vi "BSM Signal Table Save.vi"(5 "Base Ex Info":T4, 6 "Total assembly C":T1 {"Assembly Ratio 2" format="%#_3g"; "Assembly Ratio" format="%#_3g"}, 7 "BNAL Path":T2, 8 "error in":errorcluster caption="エラー入力", 9 "Save CV":T5, 10 "BC1":cluster{"B region#":i32, "Date":string}, 11 "LS Path":T3) -> (0 "error out":errorcluster)   [LabVIEW 2018]
panel:
  out "Long Signal#":i32
  out "B region#":i32
  out "L Time Profile Table":string[][](table) caption="Time Table"
  out "LS_E_J Path":path
  out "LS_E_T Path":path
  out "Time Graph":cluster{"time":dbl[], "current":dbl[]}[](graph)
  out "File F_Name":string
  out "LS_T":string
  out "Mx Right Read Seq":i32
  out "T IDX End Save":i32[](array[numeric])
  out "T IDX Start Save":i32[](array[numeric])
  out "CP A Table Tag":string[](array[string])
  out "CP T IDX End [n]":i32
  out "CP T IDX Start [n]":i32
  out "Time A Table Tag":string[](array[string])
  out "CP IDX End Save":i32[](array[numeric])
  out "CP IDX Start Save":i32[](array[numeric])
  out "L CP Profile Table":string[][](table) caption="CP Table"
  out "S CP IDX End [n]":i32
  out "S CP IDX Start [n]":i32
  out "Signal Tag AZ":string[](array[string])
  out "Time Profile Table":string[][](table) caption="Time Table"
  out "CP Profile Table":string[][](table) caption="CP Table"
  out "Long Signal Profile Table A":string[][](table) caption="Long Singla Profile Table"
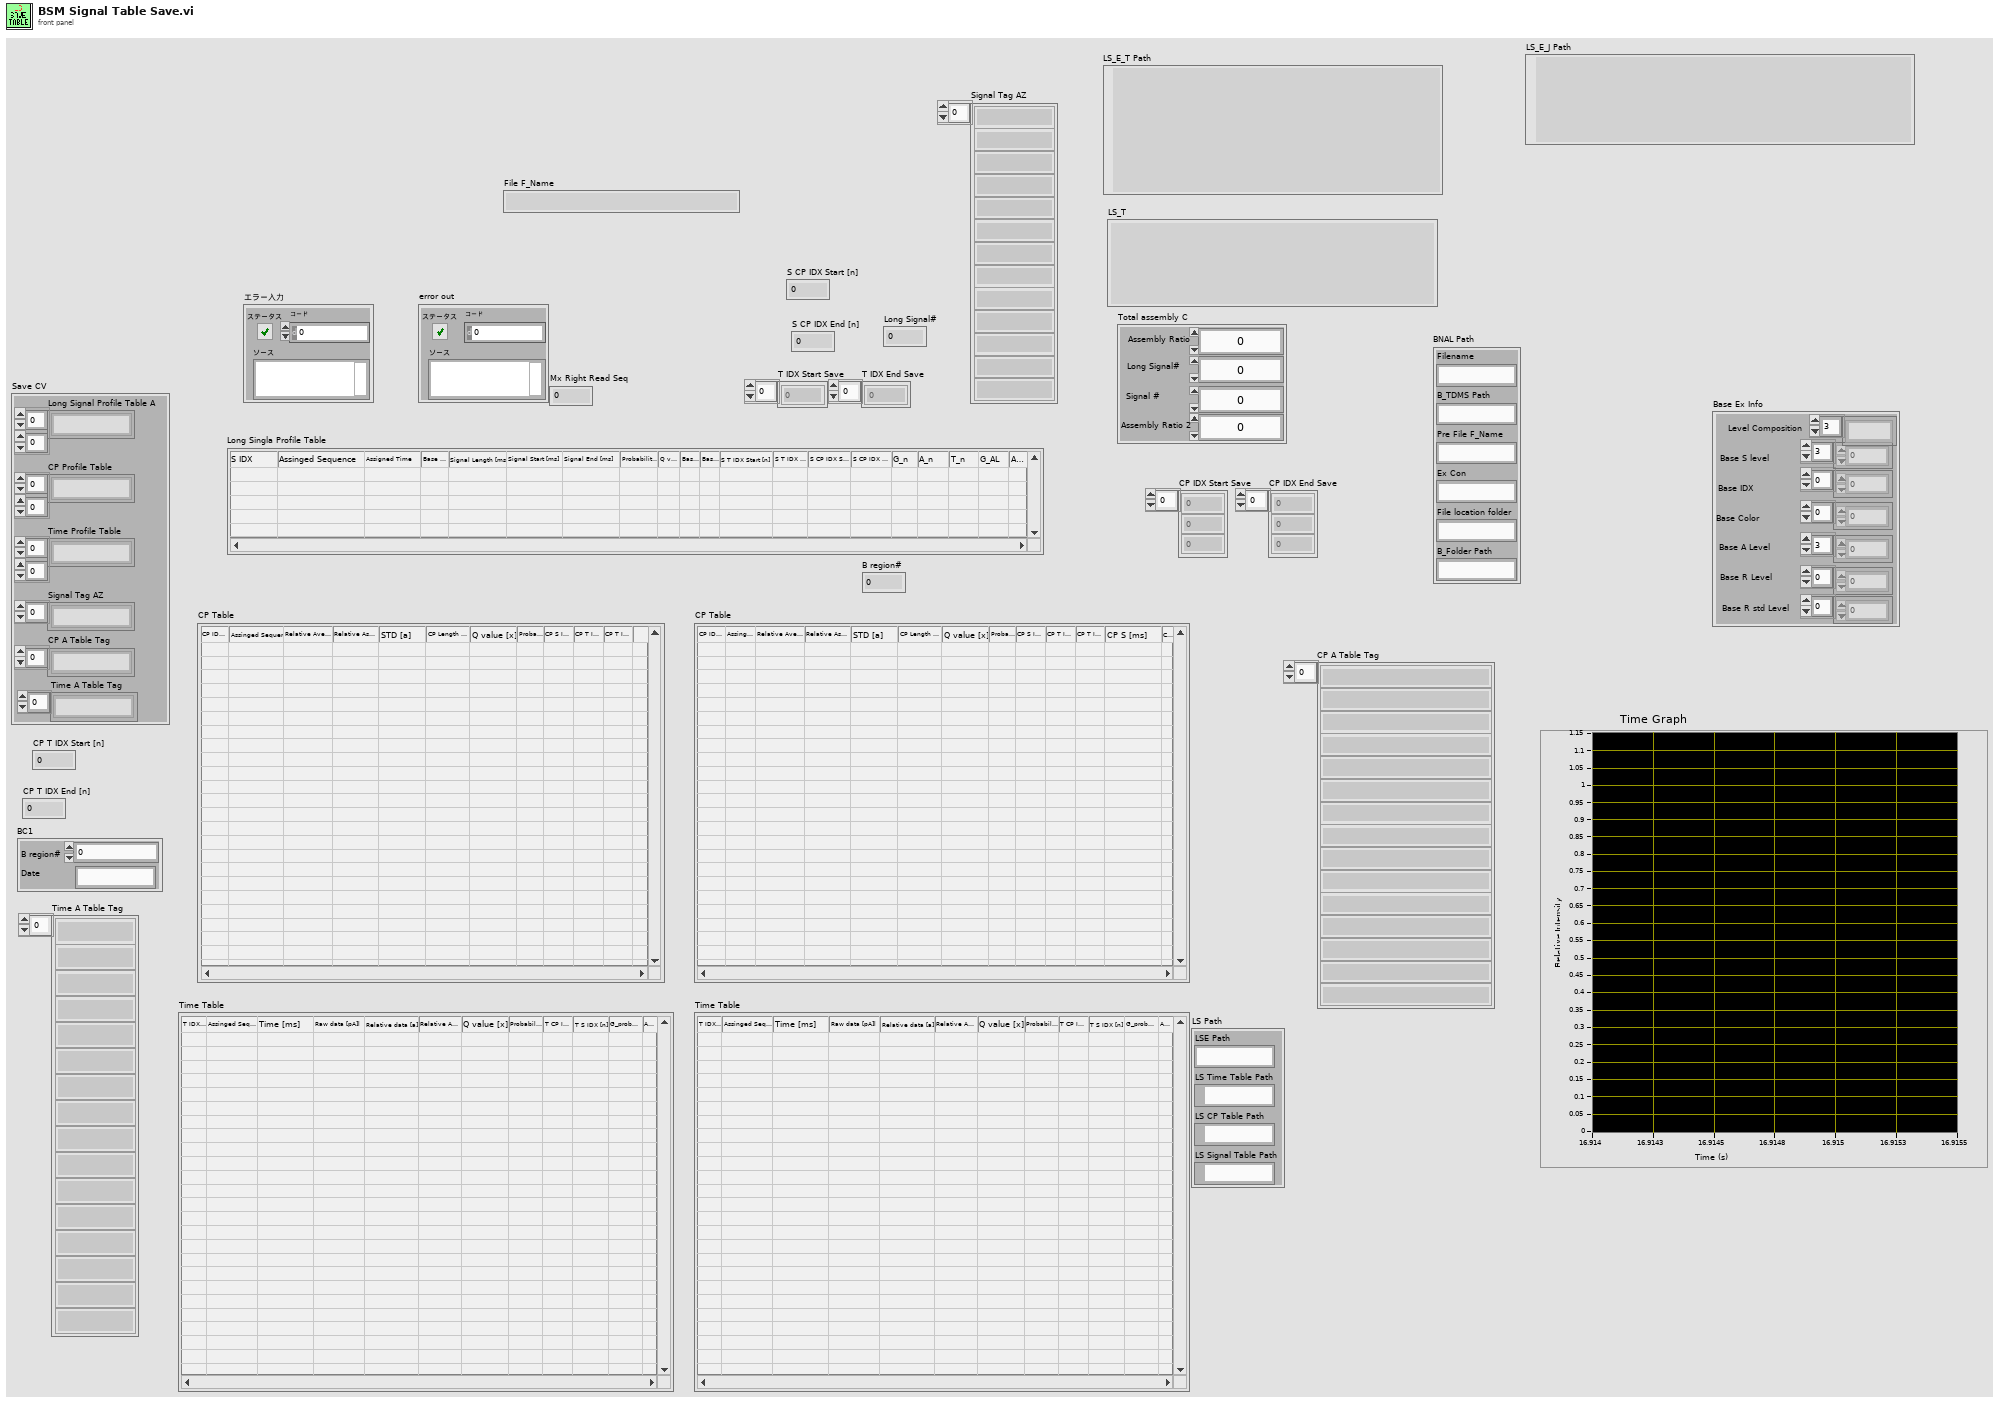
[diagram p1: front panel]
types:
  T1 = cluster{"Assembly Ratio":dbl, "Long Signal#":i32, "Signal #":i32, "Assembly Ratio 2":dbl}
  T2 = cluster{"Filename":string, "B_TDMS Path":string, "Pre File F_Name":string, "Ex Con":string, "File location folder":string, "B_Folder Path":string}
  T3 = cluster{"LSE Path":string, "LS Time Table Path":path, "LS CP Table Path":path, "LS Signal Table Path":path}
  T4 = cluster{"Level Composition":string[], "Base S level":dbl[], "Base IDX":i32[], "Base Color":u32[], "Base A Level":dbl[], "Base R Level":dbl[], "Base R std Level":dbl[]}
  T5 = cluster{"Long Signal Profile Table A ":string[][], "CP Profile Table":string[][], "Time Profile Table":string[][], "Signal Tag AZ":string[], "CP A Table Tag":string[], "Time A Table Tag":string[]}
  T6 = enum16{"open", "replace", "create", "open or create", "replace or create", "replace or create with confirmation"}
  T7 = typedef "imagedata.ctl" = cluster{"image type":i32, "image depth":i32, "image":u8[], "mask":u8[], "colors":u32[], "Rectangle":cluster{"left":i16, "top":i16, "right":i16, "bottom":i16}}
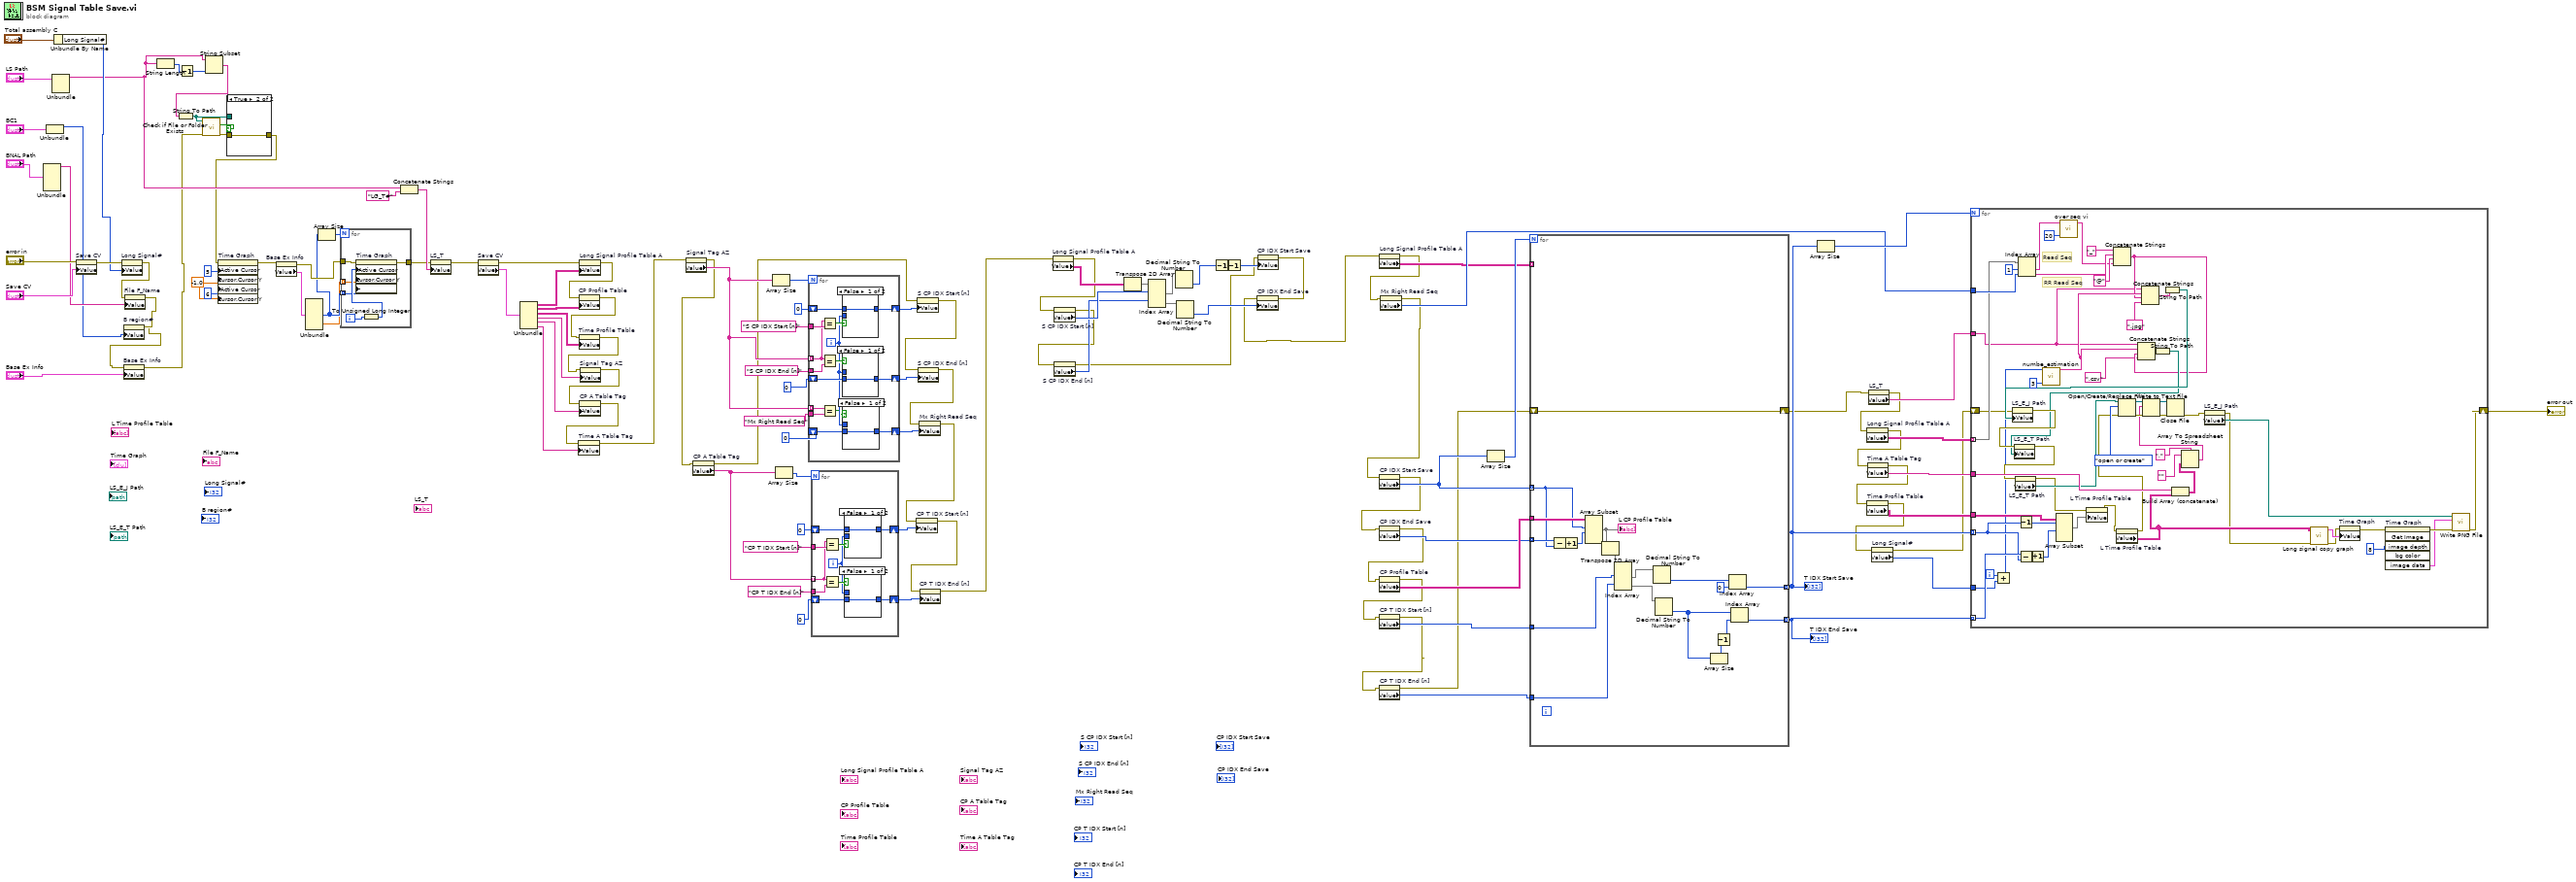
[diagram p0: block diagram]
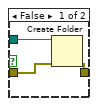
[diagram p2: hidden frame]
diagram:
  w21 = -1.0 ("カーソル.カーソル位置:カーソルY")
  n1 = Unbundle("BNAL Path") -> ("Filename"=w42:string)  [unwired: 5 out]
  n2 = Unbundle("BC1") -> ("B region#"=w34:i32)  [unwired: 1 out]
  n3 = Unbundle("LS Path") -> ("LSE Path"=w6:string)  [unwired: 3 out]
  n4 = Unbundle By Name("Total assembly C") -> ("Long Signal#"=w10:i32)
  n5 = property on="Save CV" class="Clust (strict)"(error in="error in", "Value"="Save CV") -> (error out=w36:errorcluster)  [unwired: 1 in, 1 out]
  n6 = property on="Long Signal#" class="DigNum (strict)"(error in=w36, "Value"=w10) -> (error out=w35:errorcluster)  [unwired: 1 in, 1 out]
  n7 = property on="File F_Name" class="Str"(error in=w35, "Value"=w42) -> (error out=w27:errorcluster)  [unwired: 1 in, 1 out]
  n8 = property on="B region#" class="DigNum (strict)"(error in=w27, "Value"=w34) -> (error out=w26:errorcluster)  [unwired: 1 in, 1 out]
  n9 = property on="Base Ex Info" class="Clust (strict)"(error in=w26, "Value"="Base Ex Info") -> (error out=w2:errorcluster)  [unwired: 1 in, 1 out]
  n10 = String Length(string=w6) -> (length=w5:i32)
  n11 = Decrement(x=w5) -> (x-1=w4:i32)
  n12 = String Subset(string=w6, length (rest)=w4) -> (substring=w3:string)  [unwired: 1 in]
  n13 = String To Path(string=w3) -> (path=w9:path)
  n14 = call <vilib>:"Check if File or Folder Exists.vi"("error in (no error)"=w2, "path"=w9) -> ("error out"=w7:errorcluster, "file or folder exists?"=w8:bool)  [unwired: 7 in, 1 out]
  n15 = case shown="True" w8 {
    tunnel: w9 -> [w124 _]
    tunnel: w7 -> [w123 w125]
    tunnel: [w122 w125] -> w1
    frame False {
      n16 = Create Folder(path (use dialog)=w124, error in=w123) -> (error out=w122:errorcluster)  [unwired: 1 in, 2 out]
    }
    frame True {
    }
  }
  n17 = property on="Time Graph" class="XYGraph (strict)"(error in=w1, "Active Cursor"=u32 5 ("アクティブカーソル"), "Cursor.Cursor Y"=w21, "Active Cursor"=u32 6 ("アクティブカーソル"), "Cursor.Cursor Y"=w21) -> (error out=w13:errorcluster)  [unwired: 1 in, 1 out]
  n18 = property on="Base Ex Info" class="Clust (strict)"(error in=w13) -> (error out=w17:errorcluster, "Value"=w18:T4)  [unwired: 1 in, 1 out]
  n19 = Unbundle(w18) -> ("Base Color"=w15:u32[], "Base R Level"=w14:dbl[])  [unwired: 5 out]
  n20 = Array Size(array=w15) -> (size(s)=w16:i32)
  n21 = for {
    N: w16 -> [_]
    tunnel: w17 -> [w131]
    tunnel: [w130] -> w12
    tunnel: w14 -> [w127] mode=indexing
    tunnel: w15 -> [w126] mode=indexing
    i -> [w129]
    n22 = To Unsigned Long Integer(number=w129) -> (unsigned 32bit integer=w128:u32)
    n23 = property on="Time Graph" class="XYGraph (strict)"(error in=w131, "Active Cursor"=w128, "Cursor.Cursor Y"=w127, "Cursor.Cursor Color"=w126) -> (error out=w130:errorcluster)  [unwired: 1 in, 1 out]
  }
  n24 = Concatenate Strings(w6, "LG_T#" ("文字列")) -> (w19:string)
  n25 = property on="LS_T" class="Str"(error in=w12, "Value"=w19) -> (error out=w20:errorcluster)  [unwired: 1 in, 1 out]
  n26 = property on="Save CV" class="Clust (strict)"(error in=w20) -> (error out=w40:errorcluster, "Value"=w92:T5)  [unwired: 1 in, 1 out]
  n27 = Unbundle(w92) -> ("Long Signal Profile Table A"=w80:string[][], "CP Profile Table"=w83:string[][], "Time Profile Table"=w86:string[][], "Signal Tag AZ"=w81:string[], "CP A Table Tag"=w88:string[], "Time A Table Tag"=w91:string[])
  n28 = property on="Long Signal Profile Table A" class="Tbl (strict)"(error in=w40, "Value"=w80) -> (error out=w79:errorcluster)  [unwired: 1 in, 1 out]
  n29 = property on="CP Profile Table" class="Tbl (strict)"(error in=w79, "Value"=w83) -> (error out=w78:errorcluster)  [unwired: 1 in, 1 out]
  n30 = property on="Time Profile Table" class="Tbl (strict)"(error in=w78, "Value"=w86) -> (error out=w77:errorcluster)  [unwired: 1 in, 1 out]
  n31 = property on="Signal Tag AZ" class="Arr (strict)"(error in=w77, "Value"=w81) -> (error out=w76:errorcluster)  [unwired: 1 in, 1 out]
  n32 = property on="CP A Table Tag" class="Arr (strict)"(error in=w76, "Value"=w88) -> (error out=w75:errorcluster)  [unwired: 1 in, 1 out]
  n33 = property on="Time A Table Tag" class="Arr (strict)"(error in=w75, "Value"=w91) -> (error out=w63:errorcluster)  [unwired: 1 in, 1 out]
  n34 = property on="Signal Tag AZ" class="Arr (strict)"(error in=w63) -> (error out=w62:errorcluster, "Value"=w73:string[])  [unwired: 1 in, 1 out]
  n35 = property on="CP A Table Tag" class="Arr (strict)"(error in=w62) -> (error out=w61:errorcluster, "Value"=w87:string[])  [unwired: 1 in, 1 out]
  n36 = Array Size(array=w73) -> (size(s)=w108:i32)
  n37 = Array Size(array=w87) -> (size(s)=w107:i32)
  n38 = for {
    N: w108 -> [_]
    tunnel: w73 -> [w143] mode=indexing
    tunnel: "S CP IDX Start [n]" -> [w146]
    tunnel: "S CP IDX End [n]" -> [w142]
    shift-right: [w145] -> w68
    shift-left: 0 -> [w138]
    shift-right: [w139] -> w67
    shift-left: 0 -> [w140]
    tunnel: "Mx Right Read Seq" -> [w137]
    tunnel: w73 -> [w136] mode=indexing
    shift-right: [w134] -> w66
    shift-left: 0 -> [w133]
    i -> [w135]
    n39 = Equal?(x=w143, y=w146) -> (x = y?=w144:bool)
    n40 = Equal?(x=w143, y=w142) -> (x = y?=w141:bool)
    n41 = Equal?(x=w136, y=w137) -> (x = y?=w132:bool)
    n42 = case shown="False" w144 {
      tunnel: w135 -> [_ w152]
      tunnel: [w151 w152] -> w145
      tunnel: w138 -> [w151 _]
      frame False {
      }
      frame True {
      }
    }
    n43 = case shown="False" w141 {
      tunnel: w140 -> [w149 _]
      tunnel: [w149 w150] -> w139
      tunnel: w135 -> [_ w150]
      frame False {
      }
      frame True {
      }
    }
    n44 = case shown="False" w132 {
      tunnel: w133 -> [w147 _]
      tunnel: [w147 w148] -> w134
      tunnel: w135 -> [_ w148]
      frame False {
      }
      frame True {
      }
    }
  }
  n45 = for {
    N: w107 -> [_]
    tunnel: w87 -> [w159] mode=indexing
    tunnel: "CP T IDX Start [n]" -> [w162]
    tunnel: "CP T IDX End [n]" -> [w158]
    shift-right: [w161] -> w65
    shift-left: 0 -> [w153]
    shift-right: [w155] -> w64
    shift-left: 0 -> [w156]
    i -> [w154]
    n46 = Equal?(x=w159, y=w162) -> (x = y?=w160:bool)
    n47 = Equal?(x=w159, y=w158) -> (x = y?=w157:bool)
    n48 = case shown="False" w160 {
      tunnel: w154 -> [_ w166]
      tunnel: [w165 w166] -> w161
      tunnel: w153 -> [w165 _]
      frame False {
      }
      frame True {
      }
    }
    n49 = case shown="False" w157 {
      tunnel: w156 -> [w163 _]
      tunnel: [w163 w164] -> w155
      tunnel: w154 -> [_ w164]
      frame False {
      }
      frame True {
      }
    }
  }
  n50 = property on="S CP IDX Start [n]" class="DigNum (strict)"(error in=w61, "Value"=w68) -> (error out=w60:errorcluster)  [unwired: 1 in, 1 out]
  n51 = property on="S CP IDX End [n]" class="DigNum (strict)"(error in=w60, "Value"=w67) -> (error out=w59:errorcluster)  [unwired: 1 in, 1 out]
  n52 = property on="Mx Right Read Seq" class="DigNum (strict)"(error in=w59, "Value"=w66) -> (error out=w58:errorcluster)  [unwired: 1 in, 1 out]
  n53 = property on="CP T IDX Start [n]" class="DigNum (strict)"(error in=w58, "Value"=w65) -> (error out=w57:errorcluster)  [unwired: 1 in, 1 out]
  n54 = property on="CP T IDX End [n]" class="DigNum (strict)"(error in=w57, "Value"=w64) -> (error out=w51:errorcluster)  [unwired: 1 in, 1 out]
  n55 = property on="Long Signal Profile Table A" class="Tbl (strict)"(error in=w51) -> (error out=w50:errorcluster, "Value"=w74:string[][])  [unwired: 1 in, 1 out]
  n56 = property on="S CP IDX Start [n]" class="DigNum (strict)"(error in=w50) -> (error out=w49:errorcluster, "Value"=w72:i32)  [unwired: 1 in, 1 out]
  n57 = property on="S CP IDX End [n]" class="DigNum (strict)"(error in=w49) -> (error out=w48:errorcluster, "Value"=w71:i32)  [unwired: 1 in, 1 out]
  n58 = Transpose 2D Array(2D array=w74) -> (transposed array=w115:string[][])
  n59 = Index Array(array=w115, index (row) #1=w72, index (row) #2=w71) -> (element #1=w117:string[], element #2=w116:string[])  [unwired: 2 in]
  n60 = Decimal String To Number(string=w117) -> (number=w114:i32[])  [unwired: 2 in, 1 out]
  n61 = Decimal String To Number(string=w116) -> (number=w54:i32[])  [unwired: 2 in, 1 out]
  n62 = Decrement(x=w114) -> (x-1=w113:i32[])
  n63 = Decrement(x=w113) -> (x-1=w53:i32[])
  n64 = property on="CP IDX Start Save" class="Arr (strict)"(error in=w48, "Value"=w53) -> (error out=w47:errorcluster)  [unwired: 1 in, 1 out]
  n65 = property on="CP IDX End Save" class="Arr (strict)"(error in=w47, "Value"=w54) -> (error out=w37:errorcluster)  [unwired: 1 in, 1 out]
  n66 = property on="Long Signal Profile Table A" class="Tbl (strict)"(error in=w37) -> (error out=w46:errorcluster, "Value"=w56:string[][])  [unwired: 1 in, 1 out]
  n67 = property on="Mx Right Read Seq" class="DigNum (strict)"(error in=w46) -> (error out=w30:errorcluster, "Value"=w98:i32)  [unwired: 1 in, 1 out]
  n68 = property on="CP IDX Start Save" class="Arr (strict)"(error in=w30) -> (error out=w45:errorcluster, "Value"=w52:i32[])  [unwired: 1 in, 1 out]
  n69 = property on="CP IDX End Save" class="Arr (strict)"(error in=w45) -> (error out=w44:errorcluster, "Value"=w55:i32[])  [unwired: 1 in, 1 out]
  n70 = property on="CP Profile Table" class="Tbl (strict)"(error in=w44) -> (error out=w43:errorcluster, "Value"=w82:string[][])  [unwired: 1 in, 1 out]
  n71 = property on="CP T IDX Start [n]" class="DigNum (strict)"(error in=w43) -> (error out=w29:errorcluster, "Value"=w70:i32)  [unwired: 1 in, 1 out]
  n72 = property on="CP T IDX End [n]" class="DigNum (strict)"(error in=w29) -> (error out=w28:errorcluster, "Value"=w69:i32)  [unwired: 1 in, 1 out]
  n73 = Array Size(array=w52) -> (size(s)=w101:i32)
  n74 = for {
    N: w101 -> [_]
    tunnel: w52 -> [w183] mode=indexing
    tunnel: w55 -> [w184] mode=indexing
    tunnel: w82 -> [w185]
    tunnel: w70 -> [w180]
    tunnel: w69 -> [w179]
    tunnel: [w173] -> w105 mode=indexing
    tunnel: [w169] -> w104 mode=indexing
    shift-right: [w167] -> w24
    shift-left: w28 -> [w167]
    tunnel: w56 -> [_] mode=indexing
    n75 = Subtract(x=w184, y=w183) -> (x-y=w182:i32)
    n76 = Increment(x=w182) -> (x+1=w181:i32)
    n77 = Array Subset(array=w185, index (row)=w183, length (row)=w181) -> (w168:string[][])  [unwired: 2 in]
    "L CP Profile Table" <- w168
    n78 = Transpose 2D Array(2D array=w168) -> (transposed array=w176:string[][])
    n79 = Index Array(array=w176, index (row) #1=w180, index (row) #2=w179) -> (element #1=w178:string[], element #2=w177:string[])  [unwired: 2 in]
    n80 = Decimal String To Number(string=w178) -> (number=w175:i32[])  [unwired: 2 in, 1 out]
    n81 = Decimal String To Number(string=w177) -> (number=w172:i32[])  [unwired: 2 in, 1 out]
    n82 = Array Size(array=w172) -> (size(s)=w171:i32)
    n83 = Decrement(x=w171) -> (x-1=w170:i32)
    n84 = Index Array(array=w175, index=0 ("指標")) -> (element=w173:i32)
    n85 = Index Array(array=w172, index=w170) -> (element=w169:i32)
  }
  "T IDX Start Save" <- w105
  "T IDX End Save" <- w104
  n86 = Array Size(array=w105) -> (size(s)=w106:i32)
  n87 = property on="LS_T" class="Str"(error in=w24) -> (error out=w95:errorcluster, "Value"=w97:string)  [unwired: 1 in, 1 out]
  n88 = property on="Long Signal Profile Table A" class="Tbl (strict)"(error in=w95) -> (error out=w89:errorcluster, "Value"=w96:string[][])  [unwired: 1 in, 1 out]
  n89 = property on="Time A Table Tag" class="Arr (strict)"(error in=w89) -> (error out=w84:errorcluster, "Value"=w90:string[])  [unwired: 1 in, 1 out]
  n90 = property on="Time Profile Table" class="Tbl (strict)"(error in=w84) -> (error out=w32:errorcluster, "Value"=w85:string[][])  [unwired: 1 in, 1 out]
  n91 = property on="Long Signal#" class="DigNum (strict)"(error in=w32) -> (error out=w31:errorcluster, "Value"=w33:i32)  [unwired: 1 in, 1 out]
  n92 = for {
    N: w106 -> [_]
    tunnel: w105 -> [w239] mode=indexing
    tunnel: w104 -> [w240] mode=indexing
    tunnel: w85 -> [w242]
    shift-right: [w190] -> w103
    shift-left: w31 -> [w209]
    tunnel: w90 -> [w225]
    tunnel: w98 -> [w220]
    tunnel: w97 -> [w196]
    tunnel: w96 -> [w216] mode=indexing
    tunnel: w33 -> [w200]
    i -> [w230]
    # "RR Read Seq"
    # "Read Seq"
    n93 = Add(x=w230, y=w200) -> (x+y=w201:i32)
    n94 = Decrement(x=w239) -> (x-1=w237:i32)
    n95 = Subtract(x=w240, y=w239) -> (x-y=w241:i32)
    n96 = Index Array(array=w216, index #1=1 ("指標"), index #2=w220) -> (element #1=w188:string, element #2=w218:string)
    n97 = Increment(x=w241) -> (x+1=w238:i32)
    n98 = call "numbe_estimation.vi"("桁数"=3, "数値"=w201) -> ("数値文字列"=w223:string)  [unwired: 9 in]
    n99 = Array Subset(array=w242, index (row)=w237, length (row)=w238) -> (w208:string[][])  [unwired: 2 in]
    n100 = call "over seq vi.vi"("y"=20, "Read Seq"=w188) -> ("result seq"=w187:string)  [unwired: 9 in]
    n101 = Concatenate Strings("_" ("文字列"), w218, "@" ("文字列"), w187) -> (w198:string)
    n102 = Concatenate Strings(w196, w223, w198, ".csv" ("文字列")) -> (w232:string)
    n103 = Concatenate Strings(w196, w223, w198, ".jpg" ("文字列")) -> (w222:string)
    n104 = String To Path(string=w232) -> (path=w212:path)
    n105 = String To Path(string=w222) -> (path=w214:path)
    n106 = property on="LS_E_J Path" class="Path"(error in=w209, "Value"=w214) -> (error out=w213:errorcluster)  [unwired: 1 in, 1 out]
    n107 = property on="LS_E_T Path" class="Path"(error in=w213, "Value"=w212) -> (error out=w211:errorcluster)  [unwired: 1 in, 1 out]
    n108 = property on="LS_E_T Path" class="Path"(error in=w211) -> (error out=w207:errorcluster, "Value"=w210:path)  [unwired: 1 in, 1 out]
    n109 = property on="L Time Profile Table" class="Tbl (strict)"(error in=w207, "Value"=w208) -> (error out=w206:errorcluster)  [unwired: 1 in, 1 out]
    n110 = property on="L Time Profile Table" class="Tbl (strict)"(error in=w206) -> (error out=w205:errorcluster, "Value"=w204:string[][])  [unwired: 1 in, 1 out]
    n111 = Open/Create/Replace File(file path (use dialog)=w210, error in=w205, operation (0:open)=T6."open or create" ("操作（0:open）")) -> (refnum out=w235:refnum<file>, error out=w236:errorcluster)  [unwired: 3 in, 1 out]
    n112 = Build Array (concatenate)(w225, w204) -> (w226:string[][])
    n113 = Array To Spreadsheet String(delimiter (Tab)="," ("デリミタ（タブ）"), array=w226, 3:"" ("形式文字列")) -> (spreadsheet string=w224:string)
    n114 = Write to Text File(file (use dialog)=w235, text=w224, error in=w236) -> (refnum out=w234:refnum<file>, error out=w233:errorcluster)  [unwired: 1 in, 1 out]
    n115 = Close File(refnum=w234, error in=w233) -> (error out=w202:errorcluster)  [unwired: 1 out]
    n116 = property on="LS_E_J Path" class="Path"(error in=w202) -> (error out=w189:errorcluster, "Value"=w192:path)  [unwired: 1 in, 1 out]
    n117 = call "Long signal copy graph.vi"("エラー入力（エラーなし）"=w189, "L Time Profile Table"=w204) -> ("エラー出力"=w203:errorcluster, "Time Graph"=w215:cluster{"time":dbl[], "current":dbl[]}[])  [unwired: 8 in]
    n118 = property on="Time Graph" class="XYGraph (strict)"(error in=w203, "Value"=w215) -> (error out=w191:errorcluster)  [unwired: 1 in, 1 out]
    n119 = invoke on="Time Graph" class="XYGraph （指定）" method="Get Image"(error in=w191, "image depth"=8 ("画像深度")) -> (error out=w195:errorcluster, "image data"=w193:T7)  [unwired: 4 in, 4 out]
    n120 = call <vilib>:"Write PNG File.vi"("error in (no error)"=w195, "image data"=w193, "path to PNG file"=w192) -> ("error out"=w190:errorcluster)  [unwired: 7 in, 1 out]
  }
  "error out" <- w103
